vi "KnifeEdgeExpt.vi"(7 "Rep. Rate (Hz)":dbl=1000.0 min=0.0 max=34.0, 10 "Start Position":dbl[](array[numeric]) min=0.0 max=34.0) -> (0 "SDG_Ctrl":bool, 1 "start/end points":cluster{dbl, dbl, dbl}[][](array[cluster]), 2 "Canceled":bool, 3 "Angle_Incident":dbl caption="Incident\nAngle (deg)", 4 "X/Y (T:Y)":bool=TRUE, 5 "ImageParameter":T1, 6 "w_fit_init.":dbl[](array[numeric])=[0.0, 1.0, 10.0, 0.01], 8 "z0_fit_init.":dbl[](array[numeric])=[0.01, 10.0, 1.0])   [LabVIEW 2013]
uses:
  ImagingMS/ImageConvPara_3d.ctl
  <vilib>/Native 3D Graph/xcontrol/3DPC_SurfacePlot.xctl
panel:
  in  "w_fit_initial values":dbl[](array[numeric])=[0.0, 1.0, 10.0, 0.01]
  in  "z0_fit_initial values":dbl[](array[numeric])=[0.01, 10.0, 1.0]
  in  "MainAixalStepWidth":dbl=0.01 caption="Y StepWidth"
  out "3D Graph":refnum<class "Base Datatype.lvclass">[](xcontrol)
  in  "x ? y":bool=TRUE
  in  "IncidentAngle":dbl caption="Incident\nAngle (deg)"
  in  "SDG Ctrl?":bool=TRUE
  out "Estimated Time (min)":dbl min=0.0 max=34.0
  in  "Average":i32=10 min=20 max=1000 step=20
  in  "Apply":bool
  in  "Cancel":bool
  in  "Run":bool
  out "2ndAxialSize":dbl caption="Z Size (mm)" min=0.0 max=34.0
  out "MainAxialSize":dbl caption="X Size (mm)" min=0.0 max=34.0
  in  "2ndAxialSteps":i32=20 caption="Z Steps" min=0 max=65535 step=1
  in  "MainAxialSize":dbl=0.5 caption="Y Size" min=0.0 max=34.0
  in  "2ndAxialStepWidth":dbl=0.04 caption="Z StepWidth" min=0.0 max=34.0
  # "Unit is mm always."
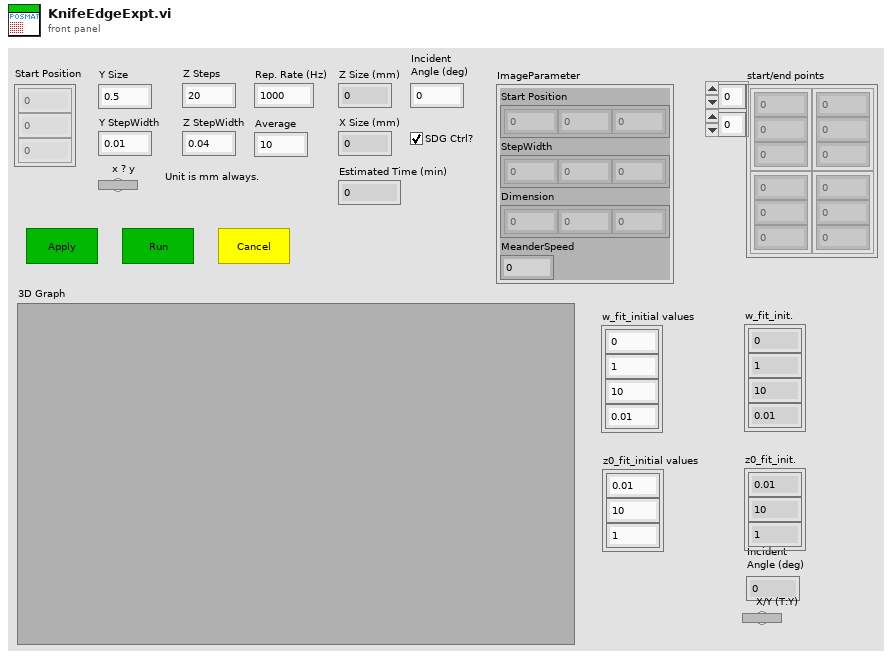
[diagram p1: front panel]
types:
  T1 = typedef "ImageConvPara_3d.ctl" = cluster{"Start Position":dbl[], "StepWidth":dbl[], "Dimension":i32[], "MeanderSpeed":dbl}
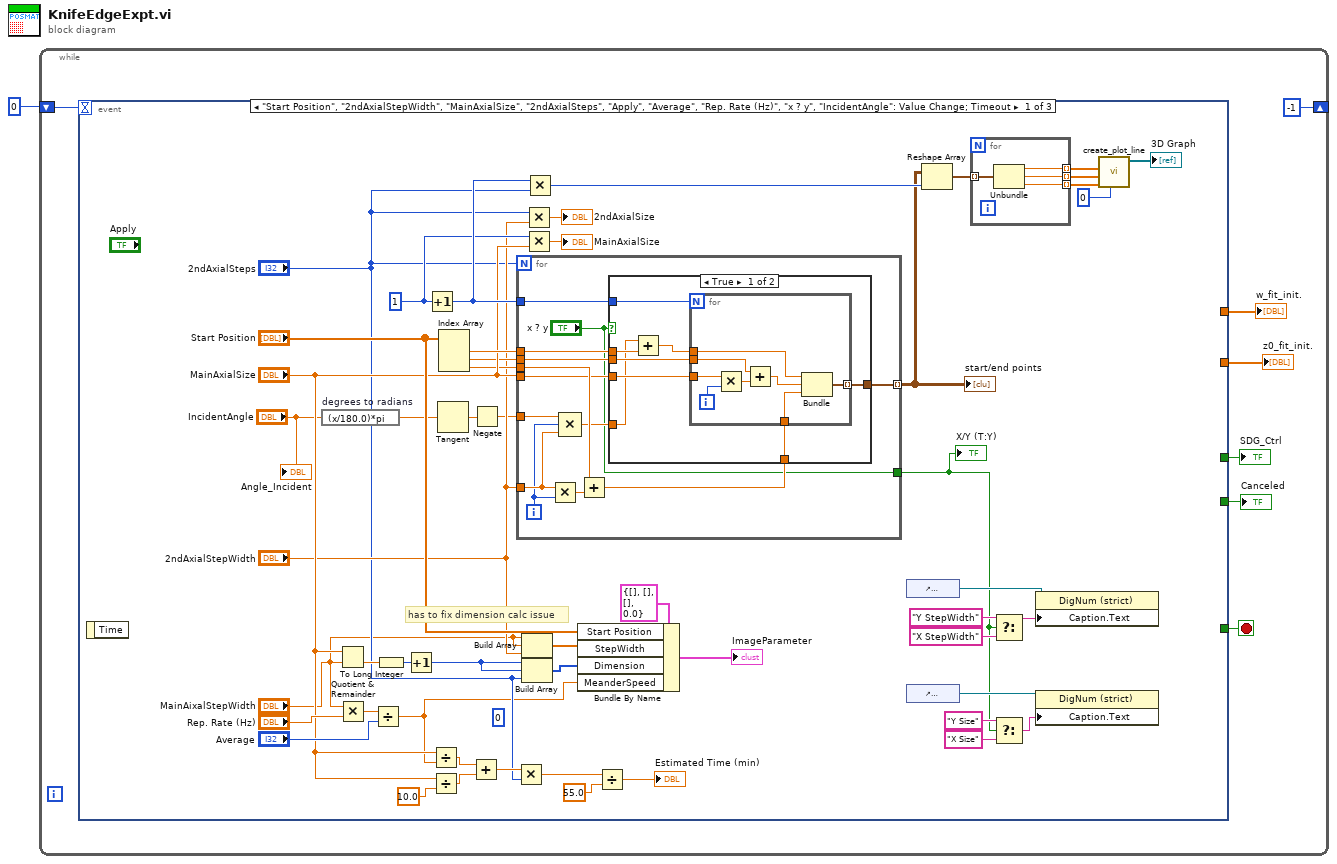
[diagram p0: block diagram]
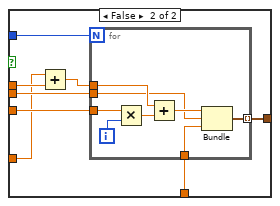
[diagram p2: hidden frame]
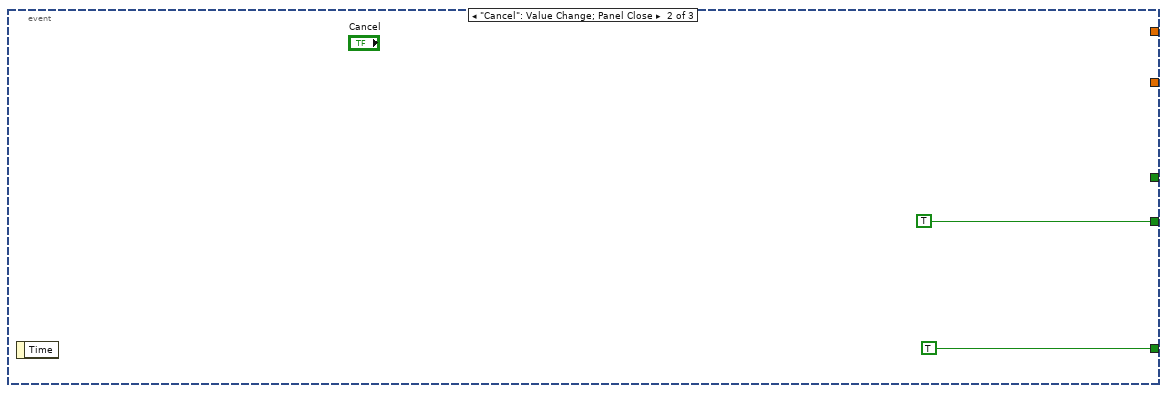
[diagram p3: hidden frame]
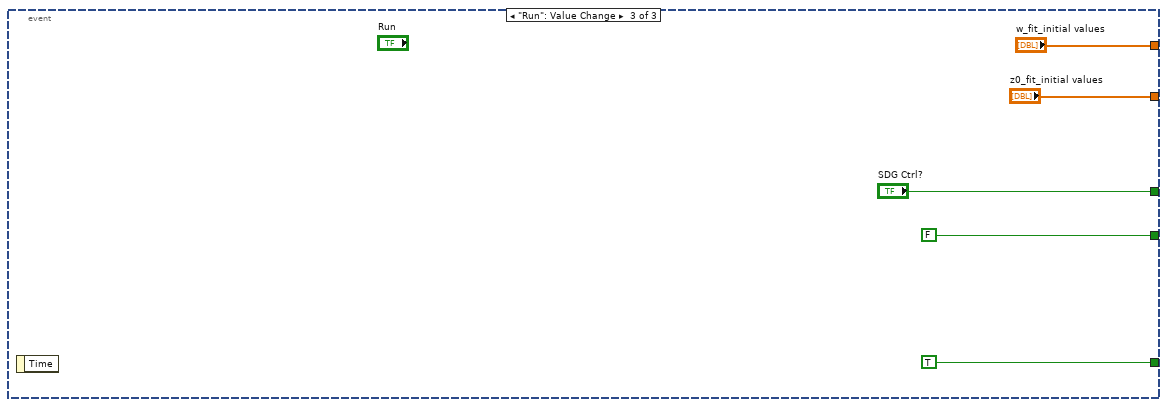
[diagram p4: hidden frame]
diagram:
  n1 = while {
    shift-right: [-1] -> _
    shift-left: 0 -> [w5]
    stop <- w8 stop-if-true
    n2 = event shown="[0] \"Start Position\", \"2ndAxialStepWidth\", \"MainAxialSize\", \"2ndAxialSteps\", \"Apply\", \"Average\", \"Rep. Rate (Hz)\", \"x ? y\", \"IncidentAngle\": Value Change;  Timeout" {
      selector: _ -> [_ _ _]
      dyn-events: _ -> [_ _ _]
      timeout: w5 -> [_ _ _]
      tunnel: [_ TRUE TRUE] -> w8
      tunnel: [_ TRUE ("Canceled") FALSE ("Canceled")] -> w7
      tunnel: [_ _ "SDG Ctrl?"] -> w6
      tunnel: [_ _ "w_fit_initial values"] -> w3
      tunnel: [_ _ "z0_fit_initial values"] -> w2
      event "Start Position", "2ndAxialStepWidth", "MainAxialSize", "2ndAxialSteps", "Apply", "Average", "Rep. Rate (Hz)", "x ? y", "IncidentAngle": Value Change; Timeout {
        (unwired) 0 ("element")
        w54 = 1
        # "has to fix dimension calc issue"
        n3 = event-data() -> ()  [unwired: 1 in, 1 out]
        n4 = expression code="(x/180.0)*pi" "degrees to radians"("IncidentAngle") -> (w28:dbl)
        n5 = Quotient & Remainder(x="MainAxialSize", y="MainAixalStepWidth") -> (floor(x/y)=w47:dbl)  [unwired: 1 out]
        n6 = Multiply(x="MainAixalStepWidth", y="Rep. Rate (Hz)") -> (x*y=w20:dbl)
        n7 = Divide(x=w20, y="Average") -> (x/y=w31:dbl)
        n8 = To Long Integer(number=w47) -> (32bit integer=w48:i32)
        n9 = Increment(x=w48) -> (x+1=w11:i32)
        n10 = Increment(x=w54) -> (x+1=w55:i32)
        n11 = Divide(x="MainAxialSize", y=w31) -> (x/y=w43:dbl)
        n12 = Divide(x="MainAxialSize", y=10.0) -> (x/y=w42:dbl)
        n13 = Tangent(1:w28) -> (0:w30:dbl)
        n14 = Index Array(array="Start Position") -> (element #1=w59:dbl, element #2=w35:dbl, element #3=w36:dbl)  [unwired: 3 in]
        n15 = Add(x=w43, y=w42) -> (x+y=w41:dbl)
        n16 = Negate(x=w30) -> (-x=w29:dbl)
        n17 = Multiply(x=w41, y="2ndAxialSteps") -> (x*y=w40:dbl)
        n18 = for {
          N: "2ndAxialSteps" -> [_]
          tunnel: w36 -> [w72]
          tunnel: "2ndAxialStepWidth" -> [w67]
          tunnel: "MainAxialSize" -> [w71]
          tunnel: w55 -> [w74]
          tunnel: [w73] -> w34 mode=indexing
          tunnel: w29 -> [w68]
          tunnel: w59 -> [w70]
          tunnel: w35 -> [w69]
          tunnel: ["x ? y"] -> w9
          i -> [w66]
          n19 = Multiply(x=w67, y=w66) -> (x*y=w76:dbl)
          n20 = Compound Arithmetic op=MULTIPLY(w68, w66, w67) -> (w65:dbl)
          n21 = Add(x=w72, y=w76) -> (x+y=w75:dbl)
          n22 = case shown="True" "x ? y" {
            tunnel: w75 -> [w84 w100]
            tunnel: w74 -> [w83 w99]
            tunnel: [w82 w98] -> w73
            tunnel: w71 -> [w81 w97]
            tunnel: w70 -> [w79 w95]
            tunnel: w69 -> [w80 w96]
            tunnel: w65 -> [w77 w93]
            frame True {
              n23 = Add(x=w77, y=w79) -> (x+y=w78:dbl)
              n24 = for {
                N: w83 -> [_]
                tunnel: w81 -> [w90]
                tunnel: w78 -> [w85]
                tunnel: w84 -> [w88]
                tunnel: [w89] -> w82 mode=indexing
                tunnel: w80 -> [w87]
                i -> [w91]
                n25 = Multiply(x=w90, y=w91) -> (x*y=w92:dbl)
                n26 = Add(x=w87, y=w92) -> (x+y=w86:dbl)
                n27 = Bundle(w85, w86, w88) -> (w89:cluster{dbl, dbl, dbl})  [unwired: 1 in]
              }
            }
            frame False {
              n28 = Add(x=w93, y=w95) -> (x+y=w94:dbl)
              n29 = for {
                N: w99 -> [_]
                tunnel: w97 -> [w106]
                tunnel: w94 -> [w102]
                tunnel: w100 -> [w103]
                tunnel: [w105] -> w98 mode=indexing
                tunnel: w96 -> [w101]
                i -> [w107]
                n30 = Multiply(x=w106, y=w107) -> (x*y=w108:dbl)
                n31 = Add(x=w102, y=w108) -> (x+y=w104:dbl)
                n32 = Bundle(w104, "X StepWidth"=w101, w103) -> (w105:cluster{dbl, "X StepWidth":dbl, dbl})  [unwired: 1 in]
              }
            }
          }
        }
        "start/end points" <- w34
        "X/Y (T:Y)" <- w9
        n33 = Build Array("MainAixalStepWidth", "MainAixalStepWidth", "2ndAxialStepWidth") -> (w51:dbl[])
        n34 = Build Array(w11, w11, "2ndAxialSteps") -> (w50:i32[])
        n35 = Multiply(x="2ndAxialSteps", y="2ndAxialStepWidth") -> (x*y=→"2ndAxialSize":dbl)
        n36 = Multiply(x=w54, y="MainAxialSize") -> (x*y=→"MainAxialSize":dbl)
        n37 = Multiply(x=w55, y="2ndAxialSteps") -> (x*y=w56:i32)
        n38 = Bundle By Name(cluster=T1 {"Start Position"=[], "StepWidth"=[], "Dimension"=[], "MeanderSpeed"=0.0} ("ImageParameter"), "Start Position"="Start Position", "StepWidth"=w51, "Dimension"=w50, "MeanderSpeed"=w31) -> (→"ImageParameter":T1)
        n39 = Divide(x=w40, y=55.0) -> (x/y=→"Estimated Time (min)":dbl)
        n40 = control-ref of="MainAixalStepWidth"() -> (w19:refnum<vi>)
        n41 = control-ref of="MainAxialSize"() -> (w18:refnum<vi>)
        n42 = Reshape Array(w34, w56) -> (w21:cluster{dbl, "X StepWidth":dbl, dbl}[])
        n43 = for {
          tunnel: w21 -> [w63] mode=indexing
          tunnel: [w62] -> w24 mode=indexing
          tunnel: [w61] -> w25 mode=indexing
          tunnel: [w60] -> w26 mode=indexing
          n44 = Unbundle(w63) -> (w62:dbl, "X StepWidth"=w61:dbl, w60:dbl)
        }
        n45 = Select(t="Y StepWidth" ("Label.Text"), s=w9, f="X StepWidth" ("Label.Text")) -> (s? t:f=w17:string)
        n46 = Select(t="Y Size" ("Label.Text"), s=w9, f="X Size" ("Label.Text")) -> (s? t:f=w12:string)
        n47 = property class="DigNum (strict)"(reference=w19, "Caption.Text"=w17) -> ()  [unwired: 1 in, 2 out]
        n48 = property class="DigNum (strict)"(reference=w18, "Caption.Text"=w12) -> ()  [unwired: 1 in, 2 out]
        n49 = call <vilib>:"create_plot_line.vi"("plot ID"=0, "z vector"=w26, "y vector"=w25, "x vector"=w24) -> ("plots out"=→"3D Graph":refnum<class "Base Datatype.lvclass">[])  [unwired: 1 in, 6 out]
        "Angle_Incident" <- "IncidentAngle"
      }
      event "Cancel": Value Change; Panel Close {
        n50 = event-data() -> ()  [unwired: 1 in, 1 out]
      }
      event "Run": Value Change {
        n51 = event-data() -> ()  [unwired: 1 in, 1 out]
      }
    }
    "Canceled" <- w7
    "SDG_Ctrl" <- w6
    "w_fit_init." <- w3
    "z0_fit_init." <- w2
  }
